vi "onHttpPost (Buffer).vi"(6 "timeout":i32=10000, 7 "output file":path, 8 "error in":errorcluster, 9 "buffer":string, 10 "url":string, 11 "http-method in":refnum<class "REST Client.lvclass">) -> (0 "error out":errorcluster, 1 "body":string, 2 "headers":string, 3 "http-method out":refnum<class "REST Client.lvclass">)   [LabVIEW 2020, in "REST Client.lvlib" / "REST Client.lvclass"]
uses:
  REST Client.lvclass
  REST Client.lvclass/REST Client.ctl
  http-client/http-client.lvclass
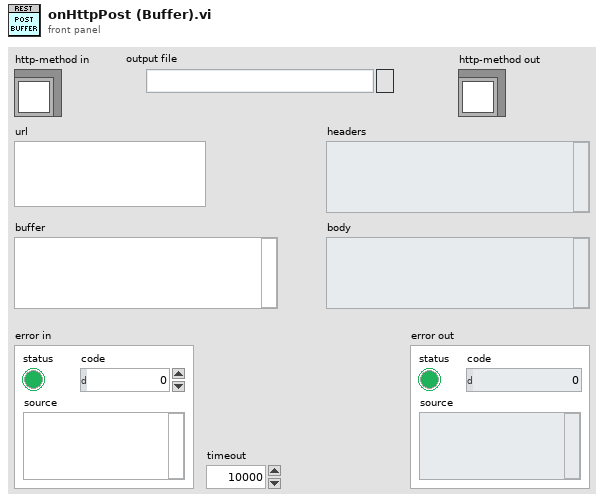
[diagram p1: front panel]
types:
  T1 = typedef "REST Client.lvlib/REST Client.lvclass/HTTP Header.ctl" = cluster{"header":T2, "value":string}
  T2 = typedef "lib_NI_Advanced HTTP Client.lvlib/Session.lvclass/Header--Combo Box.ctl" = string
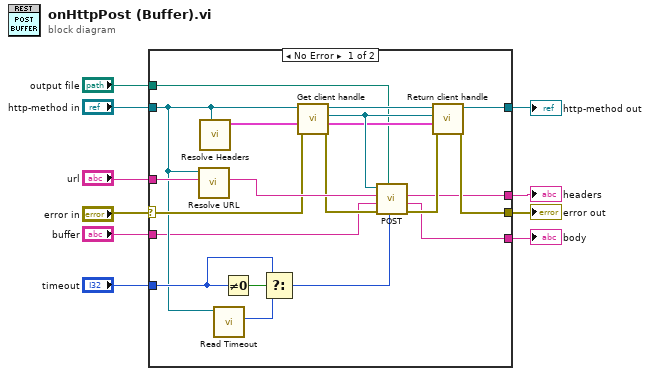
[diagram p0: block diagram]
diagram:
  n1 = case shown="No Error" "error in" {
    selector: "error in" -> [w19 w32]
    tunnel: [w15 w32] -> w6
    tunnel: [w16 w31] -> w8
    tunnel: "http-method in" -> [w18 w31]
    tunnel: "url" -> [w27 _]
    tunnel: "timeout" -> [w24 _]
    tunnel: [w14 _] -> w7
    tunnel: [w13 _] -> w5
    tunnel: "output file" -> [w12 _]
    tunnel: "buffer" -> [w11 _]
    frame No Error {
      n2 = call "Resolve URL.vi"("Path"=w27, "REST Client in"=w18) -> ("Resolved URL"=w26:string)  [unwired: 9 in]
      n3 = call "Resolve Headers.vi"("REST Client in"=w18) -> ("headers out"=w17:T1[])  [unwired: 10 in]
      n4 = call-dynamic "Read Timeout.vi"("REST Client in"=w18) -> ("Timeout"=w21:i32)  [unwired: 8 in, 2 out]
      n5 = Not Equal To 0?(x=w24) -> (x != 0?=w25:bool)
      n6 = Select(t=w24, s=w25, f=w21) -> (s? t:f=w23:i32)
      n7 = call "Get client handle.vi"("error in (no error)"=w19, "headers"=w17, "REST Client in"=w18) -> ("error out"=w22:errorcluster, "headers out"=w28:T1[], "http-client"=w29:refnum<class "http-client.lvclass">, "REST Client out"=w30:refnum<class "REST Client.lvclass">)  [unwired: 5 in]
      n8 = call "POST.vi"("timeout"=w23, "output file"=w12, "error in"=w22, "buffer"=w11, "url"=w26, "http-client in"=w29) -> ("error out"=w20:errorcluster, "body"=w13:string, "headers"=w14:string)  [unwired: 1 in, 2 out]
      n9 = call "Return client handle.vi"("error in (no error)"=w20, "headers"=w28, "http-client"=w29, "REST Client in"=w30) -> ("error out"=w15:errorcluster, "REST Client out"=w16:refnum<class "REST Client.lvclass">)  [unwired: 6 in]
    }
    frame Error {
    }
  }
  "error out" <- w6
  "http-method out" <- w8
  "headers" <- w7
  "body" <- w5
